vi "Add Multiple Arguments.vi"(9 "error in (no error)":errorcluster, 11 "error arguments":string) -> (1 "error out":errorcluster)   [LabVIEW 2019, in "Error Generation.lvlib"]
doc: "Add arguments. The format should be\n\nargument name 1 = argument data 1\nargument name 2 = argument data 2\n\nEmpty data are allowed.\nWhen there is no \"=\" for an argument, just this argument will be shown wrong.\n- - -\nCopyright (c) 2023, Merecs Engineering GmbH"
uses:
  Error Generation.lvlib
panel:
  # "Connector Pane"
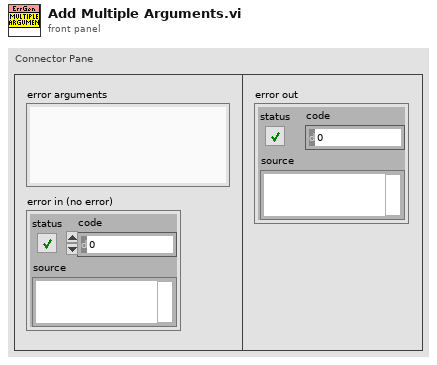
[diagram p1: front panel]
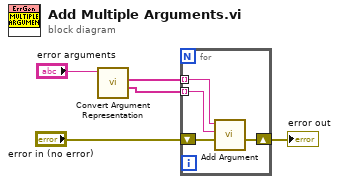
[diagram p0: block diagram]
diagram:
  n1 = call "Convert Argument Representation.vi"("error argument string"="error arguments") -> ("Data"=w4:string[], "Arguments"=w3:string[])  [unwired: 7 in, 1 out]
  n2 = for {
    shift-right: [w8] -> w2
    shift-left: "error in (no error)" -> [w9]
    tunnel: w3 -> [w7] mode=indexing
    tunnel: w4 -> [w6] mode=indexing
    n3 = call "Add Argument.vi"("error in (no error)"=w9, "argument data"=w6, "argument"=w7) -> ("error out"=w8:errorcluster)  [unwired: 8 in]
  }
  "error out" <- w2
